vi "Own20261013_AddClassFields_RefsV3.vi"() -> ()   [LabVIEW 2024]
uses:
  <resource>/Framework/Providers/MessageMakerProvider/_Message Maker/Message Maker.lvlib
panel:
  out "error out":errorcluster caption="错误输出"
  in  "Carrier Path":path
  in  "Target Path":path
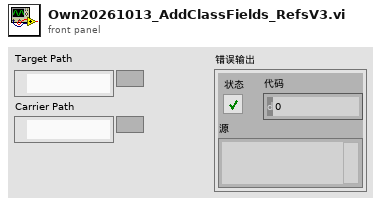
[diagram p1: front panel]
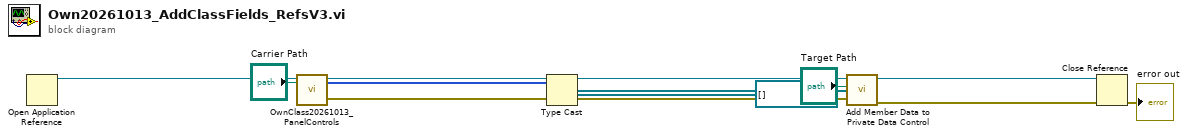
[diagram p0: block diagram]
diagram:
  n1 = Open Application Reference() -> (3:w7:refnum<vi>)  [unwired: 4 in, 1 out]
  n2 = call "OwnClass20261013_PanelControls.vi"("target_path"="Carrier Path") -> ("error out"=w6:errorcluster, "control_ids"=w4:u32[])  [unwired: 1 in]
  n3 = Type Cast(type=refnum<vi>[] [] ("Controls"), x=w4) -> (*(type *) &x=w3:refnum<vi>[])
  n4 = call <resource>:"Add Member Data to Private Data Control.vi"("AppInst"=w7, "error in (no error)"=w6, "Controls"=w3, "Target Path"="Target Path") -> ("error out"=w2:errorcluster)  [unwired: 7 in]
  n5 = Close Reference(reference=w7, error in (no error)=w2) -> (error out=→"error out":errorcluster)
